vi "UE_Hydraulic_Power_kW.vi"(1 "flow_lpm":dbl, 2 "pressure_bar":dbl) -> (0 "hydraulic_kw":dbl)   [LabVIEW 2026]
doc: "INTENT: Calculate ideal hydraulic power from pressure bar and volumetric flow L/min. INPUTS: pressure_bar (double), flow_lpm (double). OUTPUTS: hydraulic_kw (double). DESIGN CONSTRAINT: For positive differential pressure and actual volumetric flow; this is not shaft electrical power. REQUIREMENTS: SRS-F-019. No physical hardware side effects. Acceptance requires native LabVIEW compilation and behavioral testing."
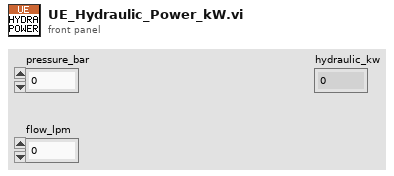
[diagram p1: front panel]
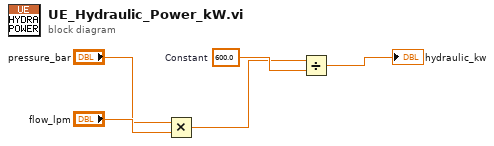
[diagram p0: block diagram]
diagram:
  w4 = 600.0  # Constant
  n1 = Multiply(x="pressure_bar", y="flow_lpm") -> (x*y=w3:dbl)
  n2 = Divide(x=w3, y=w4) -> (x/y=→"hydraulic_kw":dbl)
